vi "Update Scale List.vi"(8 "error in (no error)":errorcluster, 11 "Data Viewer in":refnum<class "Data Viewer.lvclass">) -> (0 "error out":errorcluster, 2 "Scale Name List":string[](array[string]), 3 "Data Viewer out":refnum<class "Data Viewer.lvclass">)   [LabVIEW 2020, in "Data Viewer.lvlib" / "Data Viewer.lvclass"]
uses:
  Data Viewer.lvclass
  Data Viewer.lvclass/Data Viewer.ctl
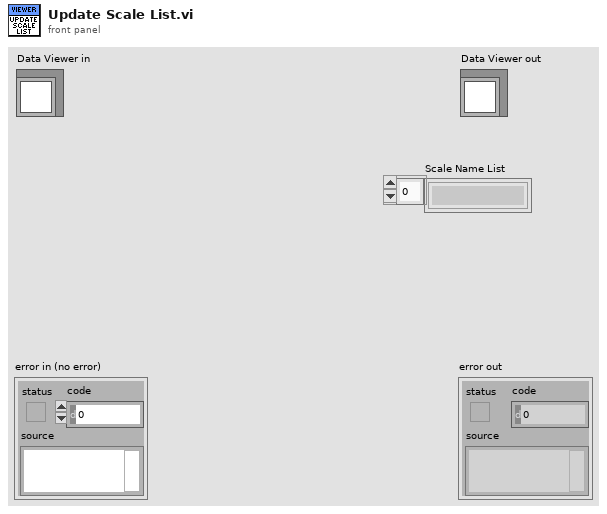
[diagram p1: front panel]
types:
  T1 = typedef "Data Viewer.lvlib/Data Viewer.lvclass/Scale Setting--cluster.ctl" = cluster{"Name":string, "Unit":string, "Color":u32, "Auto Scale":bool, "Scale Min":dbl, "Scale Max":dbl, "Scale Interval":dbl, "Show Gird":bool, "Log":bool}
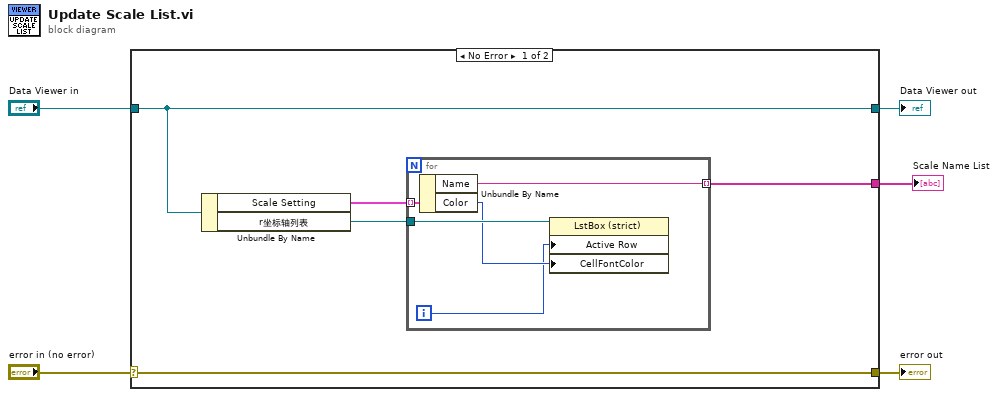
[diagram p0: block diagram]
diagram:
  n1 = case shown="No Error" "error in (no error)" {
    selector: "error in (no error)" -> [w10 w17]
    tunnel: [w10 w17] -> w4
    tunnel: [w9 w16] -> w2
    tunnel: "Data Viewer in" -> [w9 w16]
    tunnel: [w6 _] -> w1
    frame No Error {
      n2 = Unbundle By Name(w9) -> ("Scale Setting"=w7:T1[], "r坐标轴列表"=w8:refnum<vi>)
      n3 = for {
        tunnel: w8 -> [w15]
        tunnel: w7 -> [w14] mode=indexing
        tunnel: [w11] -> w6 mode=indexing
        i -> [w12]
        n4 = Unbundle By Name(w14) -> ("Name"=w11:string, "Color"=w13:u32)
        n5 = property class="LstBox (strict)"(reference=w15, "Active Row"=w12, "CellFontColor"=w13) -> ()  [unwired: 1 in, 2 out]
      }
    }
    frame Error {
    }
  }
  "error out" <- w4
  "Data Viewer out" <- w2
  "Scale Name List" <- w1
